vi "CSMs2States.vi"(9 "CSM Names":T1, 10 "States":string) -> (2 "States Out":string)   [LabVIEW 2026]
uses:
  CSM Names.ctl
  3c494fea-0774-4ab9-9bcf-ad594bcd9445.vi
  <userlib>/_NEVSTOP/Communicable State Machine(CSM)/addons/API-String-Arugments-Support/_Support/Data To API String Arguments.vi
  <userlib>/_NEVSTOP/Communicable State Machine(CSM)/Communicable State Machine.lvlib
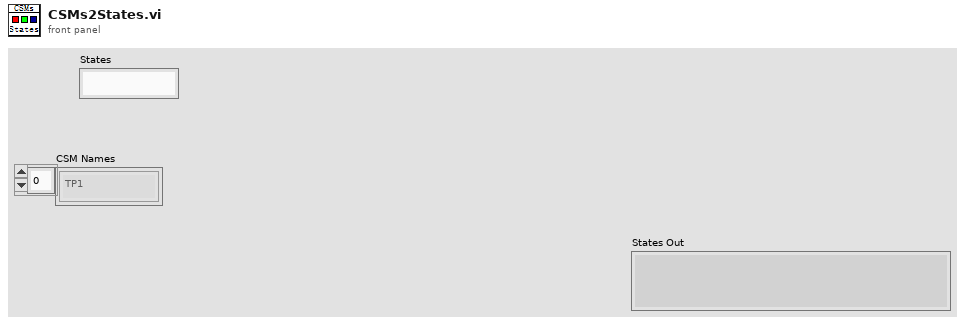
[diagram p1: front panel]
types:
  T1 = typedef "CSM Names.ctl" = string[]
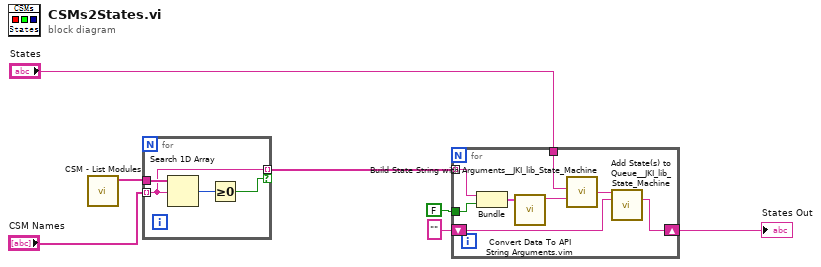
[diagram p0: block diagram]
diagram:
  n1 = call <userlib>:"CSM - List Modules.vi"() -> ("Module Names"=w6:string[])  [unwired: 10 in, 1 out]
  n2 = for {
    tunnel: "CSM Names" -> [w9] mode=indexing
    tunnel: w6 -> [w11]
    tunnel: [w9] -> w4 mode=indexing if=w8
    n3 = Search 1D Array(1D array=w11, element=w9) -> (index of element=w10:i32)  [unwired: 1 in]
    n4 = Greater Or Equal To 0?(x=w10) -> (x >= 0?=w8:bool)
  }
  n5 = for {
    tunnel: w4 -> [w14] mode=indexing
    shift-right: [w18] -> w1
    shift-left: "" ("States Out") -> [w17]
    tunnel: FALSE -> [w15]
    tunnel: "States" -> [w13]
    n6 = Bundle("Name"=w14, w15) -> (w12:cluster{"Name":string, bool})  [unwired: 1 in]
    n7 = call "Convert Data To API String Arguments.vim"("Data"=w12) -> ("API String"=w16:string)  [unwired: 7 in, 1 out]
    n8 = call <vilib>:"Build State String with Arguments__JKI_lib_State_Machine.vi"("Arguments (\"\")"=w16, "State"=w13) -> ("State with Arguments"=w19:string)  [unwired: 4 in]
    n9 = call <vilib>:"Add State(s) to Queue__JKI_lib_State_Machine.vi"("State(s) in Front (\"\")"=w19, "State(s) in (\"\")"=w17) -> ("States Out"=w18:string)  [unwired: 13 in]
  }
  "States Out" <- w1
